vi "IsWindow Wrapper Template.vi"(0 "hWnd":u64, 11 "error in":errorcluster) -> (4 "window?":bool, 15 "error out":errorcluster)   [LabVIEW 2020]
doc: "TRUE while hWnd is an existing window (of any process), through user32.dll IsWindow (stdcall, called in any thread). RemoteVI uses it to notice that a shared window of another program has closed. When error in carries an error the DLL is not called. Generated by scripts\\Build Win32 Wrappers.vi - do not edit by hand, rebuild it."
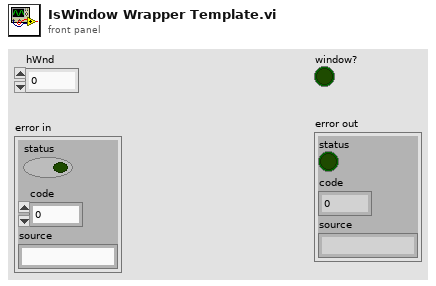
[diagram p1: front panel]
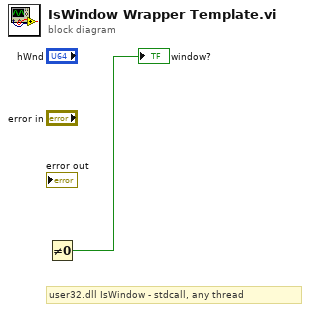
[diagram p0: block diagram]
diagram:
  # "user32.dll IsWindow - stdcall, any thread"
  n1 = Not Equal To 0?() -> (x != 0?=→"window?":bool)  [unwired: 1 in]
